vi "VIH - VI Doc Editor #2 - GenObject Properties - Read.vi"(8 "error in":errorcluster, 11 "Gen Refnum":refnum<vi>) -> (0 "error out":errorcluster, 1 "type":enum16{"<Invalid>", "Control", "Page"}(ring), 2 "Props":T1, 3 "dup Gen Refnum":refnum<vi>)   [LabVIEW 2014]
doc: "::: VI Helpeks :::\nCopyright (c) 2000-2026 Konstantin Shifershteyn. All rights reserved."
panel:
  # "VI Helpeks\nCopyright (c) 2012-2026 Konstantin Shifershteyn"
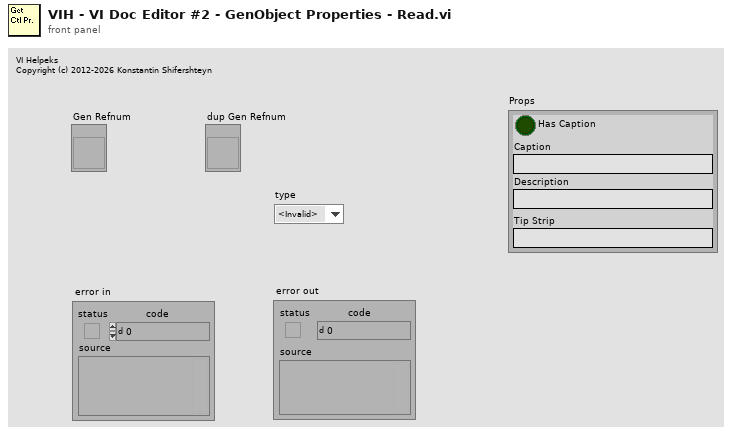
[diagram p1: front panel]
types:
  T1 = cluster{"Has Caption":bool, "Caption":string, "Description":string, "Tip Strip":string}
  T2 = cluster{"IndependentLabel":bool, "TabCaption":string, "Desc":string, "TipStrip":string}
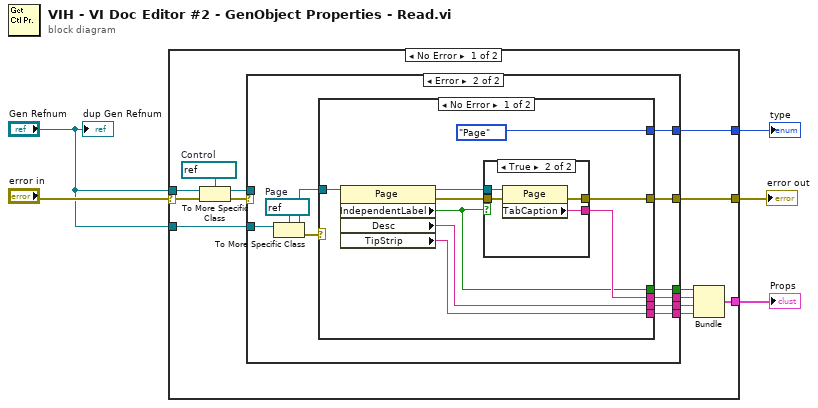
[diagram p0: block diagram]
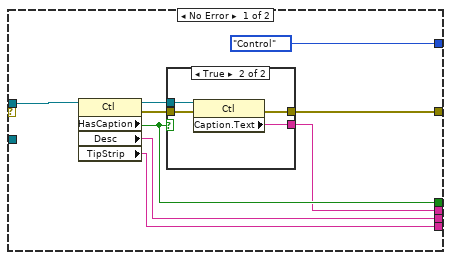
[diagram p2: hidden frame]
diagram:
  n1 = case shown="No Error" "error in" {
    selector: "error in" -> [w9 w58]
    tunnel: [w14 _] -> w5
    tunnel: [w13 w58] -> w4
    tunnel: "Gen Refnum" -> [w11 _]
    tunnel: "Gen Refnum" -> [w7 _]
    tunnel: [w6 _] -> w1
    frame No Error {
      w12 = refnum<vi> refnum  # Control
      n2 = To More Specific Class(target class=w12, reference=w11, error in=w9) -> (specific class reference=w10:refnum<vi>, error out=w8:errorcluster)
      n3 = case shown="Error" w8 {
        tunnel: [w25 w35] -> w18
        tunnel: [w24 w37] -> w17
        tunnel: [w23 w38] -> w16
        tunnel: [w22 w36] -> w15
        tunnel: [w21 w40] -> w13
        tunnel: w10 -> [w20 _]
        tunnel: w7 -> [_ w41]
        tunnel: [enum16{"<Invalid>", "Control", "Page"}."Control" ("type") w33] -> w6
        frame No Error {
          n4 = property class="Ctl"(reference=w20) -> (reference out=w27:refnum<vi>, error out=w26:errorcluster, "HasCaption"=w25:bool, "Desc"=w24:string, "TipStrip"=w23:string)  [unwired: 1 in]
          n5 = case shown="True" w25 {
            tunnel: w27 -> [_ w32]
            tunnel: w26 -> [w28 w31]
            tunnel: [_ w30] -> w22
            tunnel: [w28 w29] -> w21
            frame False {
            }
            frame True {
              n6 = property class="Ctl"(reference=w32, error in=w31) -> (error out=w29:errorcluster, "Caption.Text"=w30:string)  [unwired: 1 out]
            }
          }
        }
        frame Error {
          w42 = refnum<vi> refnum  # Page
          n7 = To More Specific Class(target class=w42, reference=w41) -> (specific class reference=w39:refnum<vi>, error out=w34:errorcluster)  [unwired: 1 in]
          n8 = case shown="No Error" w34 {
            selector: w34 -> [_ w57]
            tunnel: [w45 w57] -> w40
            tunnel: w39 -> [w51 _]
            tunnel: [w50 _] -> w38
            tunnel: [w49 _] -> w37
            tunnel: [w44 _] -> w36
            tunnel: [w43 _] -> w35
            tunnel: [enum16{"<Invalid>", "Control", "Page"}."Page" ("type") _] -> w33
            frame No Error {
              n9 = property class="Page"(reference=w51) -> (reference out=w47:refnum<vi>, error out=w46:errorcluster, "IndependentLabel"=w43:bool, "Desc"=w49:string, "TipStrip"=w50:string)  [unwired: 1 in]
              n10 = case shown="True" w43 {
                tunnel: w47 -> [_ w56]
                tunnel: w46 -> [w52 w55]
                tunnel: [w52 w54] -> w45
                tunnel: [_ w53] -> w44
                frame False {
                }
                frame True {
                  n11 = property class="Page"(reference=w56, error in=w55) -> (error out=w54:errorcluster, "TabCaption"=w53:string)  [unwired: 1 out]
                }
              }
            }
            frame Error {
            }
          }
        }
      }
      n12 = Bundle("IndependentLabel"=w18, "TabCaption"=w15, "Desc"=w17, "TipStrip"=w16) -> (w14:T2)  [unwired: 1 in]
    }
    frame Error {
    }
  }
  "error out" <- w4
  "Props" <- w5
  "type" <- w1
  "dup Gen Refnum" <- "Gen Refnum"
